vi "Initialize.vi"(0 "Universal Robot in":refnum<class "Universal Robot.lvclass">, 5 "error in (no error)":errorcluster) -> (14 "Universal Robot out":refnum<class "Universal Robot.lvclass">, 19 "error out":errorcluster)   [LabVIEW 2019, in "Universal Robot.lvclass"]
uses:
  Universal Robot.lvclass
  Universal Robot.lvclass/Universal Robot.ctl
  ProgramControlEvent.ctl
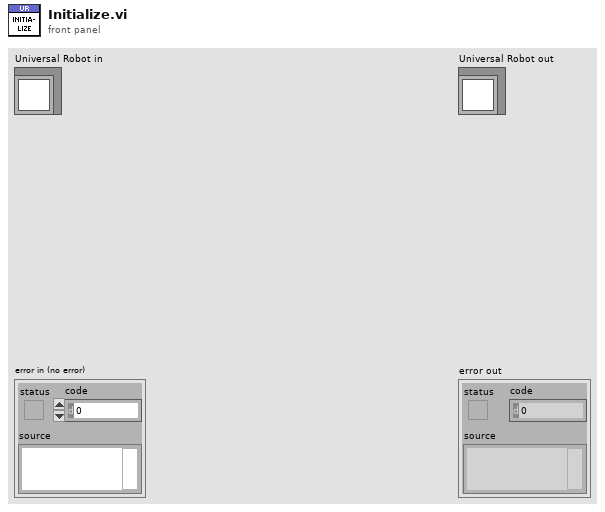
[diagram p1: front panel]
types:
  T1 = typedef "Universal Robot.lvclass/ProgramControlEvent.ctl" = enum16{"Stop", "Pause", "Resume"}
  T2 = typedef "Semaphore RefNum" = refnum<k1>
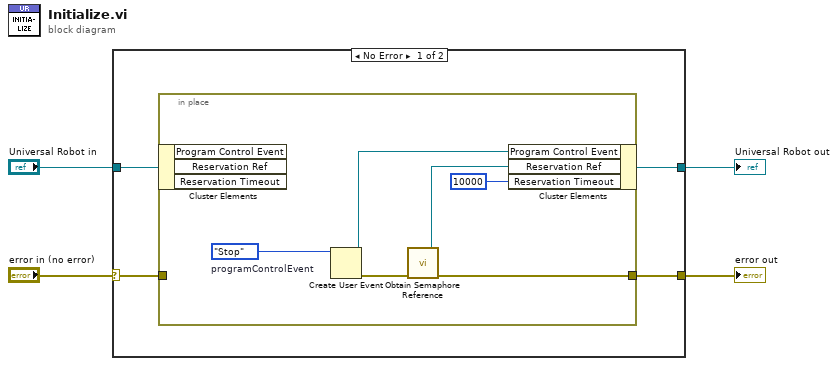
[diagram p0: block diagram]
diagram:
  n1 = case shown="No Error" "error in (no error)" {
    selector: "error in (no error)" -> [w8 w16]
    tunnel: [w7 w16] -> w3
    tunnel: [w5 w15] -> w1
    tunnel: "Universal Robot in" -> [w6 w15]
    frame No Error {
      n2 = in-place {
        in-place-border: w8 -> [_]
        in-place-border: [w11] -> w7
        w13 = ProgramControlEvent."Stop"  # programControlEvent
        n3 = in-place-cluster #1(w6) -> ()  [unwired: 3 out]
        n4 = Create User Event(user event datatype=w13) -> (user event=w14:refnum<user-event>, error out=w12:errorcluster)  [unwired: 1 in]
        n5 = call <vilib>:"Obtain Semaphore Reference.vi"("error in (no error)"=w12) -> ("error out"=w11:errorcluster, "semaphore"=w10:T2)  [unwired: 4 in, 1 out]
        n6 = in-place-cluster #1("Program Control Event"=w14, "Reservation Ref"=w10, "Reservation Timeout"=10000 ("reservationTimeout")) -> (w5:refnum<class "Universal Robot.lvclass">)
      }
    }
    frame Error {
    }
  }
  "error out" <- w3
  "Universal Robot out" <- w1
